vi "Check All Stopped.vi"(8 "error in (no error)":errorcluster, 11 "Log Manager Module in":refnum<class "Log Manager Module.lvclass">) -> (0 "error out":errorcluster, 2 "All Idle":bool, 3 "Log Manager Module out":refnum<class "Log Manager Module.lvclass">)   [LabVIEW 2020, in "VolatusData.lvlib" / "Log Manager Module.lvclass"]
uses:
  Log Manager Module.lvclass
  Log Manager Module.lvclass/Log Manager Module.ctl
  Logger State.ctl
  VolatusData.lvlib
  Logging State.ctl
  Volatus/Module/Module.lvclass
  C:/dev/lv20CE/gpack-tests/lv-volatus/Volatus/Module/Module.lvclass
  C:/dev/lv20CE/gpack-tests/lv-volatus/VolatusData/Log Manager Module/Log Manager Module.lvclass
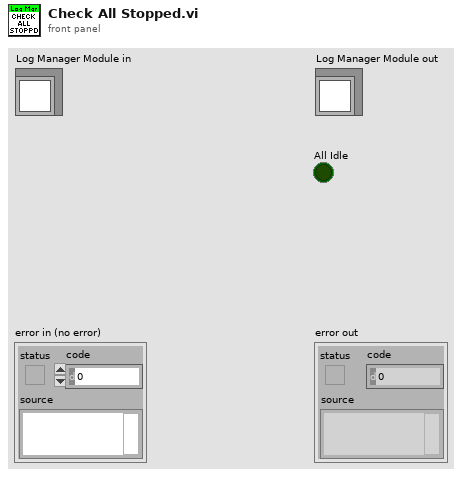
[diagram p1: front panel]
types:
  T1 = typedef "VolatusData.lvlib/Log Manager Module.lvclass/Group Info.ctl" = cluster{"Name":string, "Loggers":map{string, T2}}
  T2 = typedef "VolatusData.lvlib/Log Manager Module.lvclass/Logger.ctl" = cluster{"ID":string, "MsgQ":refnum<class "MessageQ.lvclass">, "State":T3, "Group":string}
  T3 = typedef "VolatusData.lvlib/Logger State.ctl" = enum16{"Unknown", "Idle", "Preparing", "Ready", "Logging", "Stopping"}
  T4 = typedef "VolatusData.lvlib/Logging State.ctl" = enum16{"Idle", "Starting", "Logging", "Stopping"}
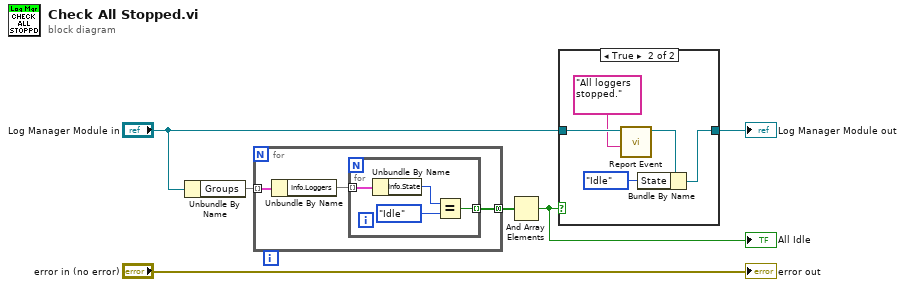
[diagram p0: block diagram]
diagram:
  n1 = Unbundle By Name("Log Manager Module in") -> ("Groups"=w3:map{string, T1})
  n2 = for {
    tunnel: [w9] -> w5 mode=concatenating
    tunnel: w3 -> [w8] mode=indexing
    n3 = Unbundle By Name(w8) -> ("Info.Loggers"=w7:map{string, T2})
    n4 = for {
      tunnel: w7 -> [w13] mode=indexing
      tunnel: [w10] -> w9 mode=indexing
      n5 = Unbundle By Name(w13) -> ("Info.State"=w12:T3)
      n6 = Equal?(x=w12, y=Logger_State."Idle") -> (x = y?=w10:bool)
    }
  }
  n7 = And Array Elements(Boolean array=w5) -> (logical AND=w4:bool)
  "All Idle" <- w4
  n8 = case shown="True" w4 {
    tunnel: "Log Manager Module in" -> [w14 w19]
    tunnel: [w14 w15] -> w1
    frame False {
    }
    frame True {
      n9 = call "Report Event.vi"("Message"="All loggers stopped.", "Module in"=w19) -> ("Module out"=w17:refnum<class "Log Manager Module.lvclass">)  [unwired: 8 in, 1 out]
      n10 = Bundle By Name(cluster=w17, "State"=Logging_State."Idle") -> (w15:refnum<class "Log Manager Module.lvclass">)
    }
  }
  "Log Manager Module out" <- w1
  "error out" <- "error in (no error)"
